vi "calculate_wildcard_filename_from_sibling_filenames.vi"(10 "shared library filename":string, 11 "sibling filenames":string[](array[string])) -> (2 "wildcard filename":string, 3 "sibling shared libraries":string[](array[string]))   [LabVIEW 2020, in "vi_package_building_extensions.lvlib" / "fix_shared_library_wildcards.lvlib"]
uses:
  fix_shared_library_wildcards.lvlib
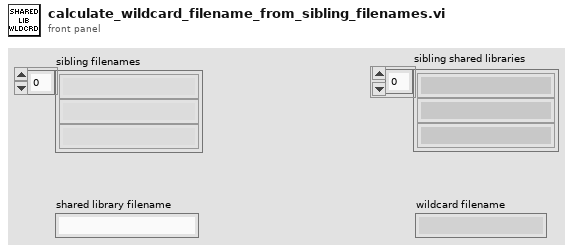
[diagram p1: front panel]
types:
  T1 = cluster{"search regex":string, "replacement":string}
  T2 = cluster{"search regex":string, "replacement":string}[]
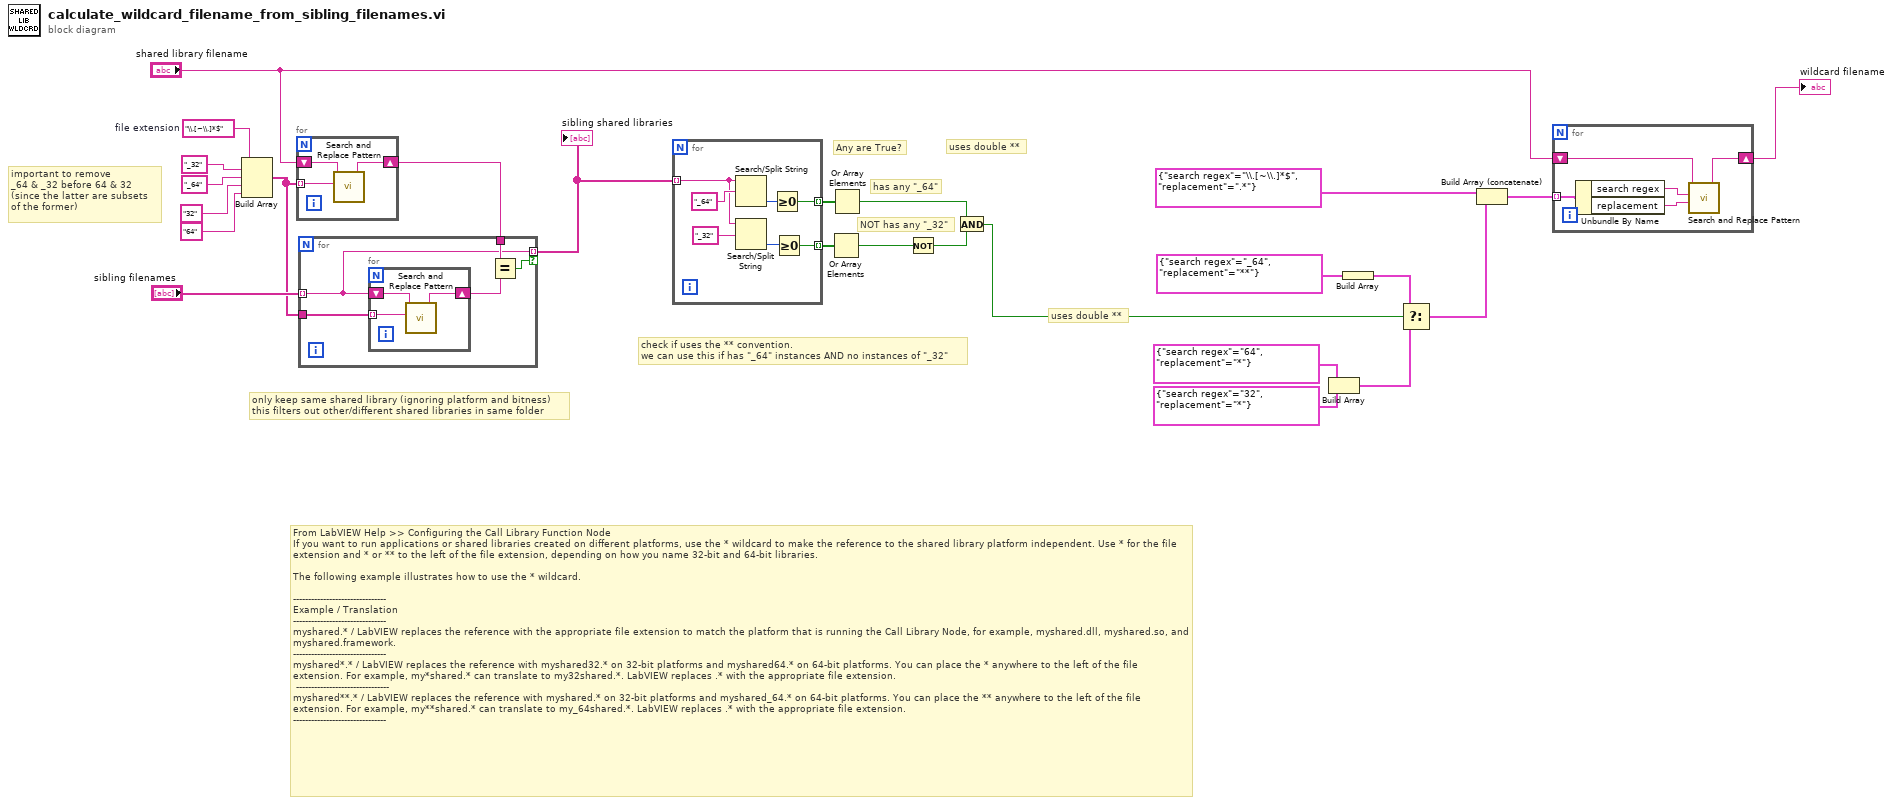
[diagram p0: block diagram]
diagram:
  w20 = "\\.[~\\.]*$"  # file extension
  # "From LabVIEW Help >> Configuring the Call Library Function Node\nIf you want to run applications or shared libraries created on different platforms, use the * wildcard to make the reference to the shared library platform independent. Use * for the file extension and * or ** to the left of the file extension, depending on how you name 32-bit and 64-bit libraries.\n\nThe following example illustrates how to use the * wildcard.\n\n-------------------------------\nExample / Translation\n-------------------------------\nmyshared.* / LabVIEW replaces the reference with the appropriate file extension to match the platform that is running the Call Library Node, for example, myshared.dll, myshared.so, and myshared.framework. \n-------------------------------\nmyshared*.* / LabVIEW replaces the reference with myshared32.* on 32-bit platforms and myshared64.* on 64-bit platforms. You can place the * anywhere to the left of the file extension. For example, my*shared.* can translate to my32shared.*. LabVIEW replaces .* with the appropriate file extension.\n -------------------------------\nmyshared**.* / LabVIEW replaces the reference with myshared.* on 32-bit platforms and myshared_64.* on 64-bit platforms. You can place the ** anywhere to the left of the file extension. For example, my**shared.* can translate to my_64shared.*. LabVIEW replaces .* with the appropriate file extension. \n-------------------------------"
  # "uses double **"
  # "only keep same shared library (ignoring platform and bitness)\nthis filters out other/different shared libraries in same folder"
  # "important to remove\n_64 & _32 before 64 & 32 (since the latter are subsets of the former)"
  # "check if uses the ** convention.\nwe can use this if has \"_64\" instances AND no instances of \"_32\""
  # "uses double **"
  # "NOT has any \"_32\""
  # "has any \"_64\""
  # "Any are True?"
  n1 = Build Array(w20, "_32", "_64", "32", "64") -> (w15:string[])
  n2 = for {
    tunnel: w15 -> [w28] mode=indexing
    shift-right: [w26] -> w14
    shift-left: "shared library filename" -> [w27]
    n3 = call <vilib>:"Search and Replace Pattern.vi"("string"=w27, "regular expression (\"\")"=w28) -> ("result string"=w26:string)  [unwired: 3 in, 1 out]
  }
  n4 = for {
    tunnel: "sibling filenames" -> [w30] mode=indexing
    tunnel: w15 -> [w33]
    tunnel: w14 -> [w32]
    tunnel: [w30] -> w13 mode=indexing if=w31
    n5 = for {
      tunnel: w33 -> [w36] mode=indexing
      shift-right: [w34] -> w29
      shift-left: w30 -> [w35]
      n6 = call <vilib>:"Search and Replace Pattern.vi"("string"=w35, "regular expression (\"\")"=w36) -> ("result string"=w34:string)  [unwired: 3 in, 1 out]
    }
    n7 = Equal?(x=w32, y=w29) -> (x = y?=w31:bool)
  }
  "sibling shared libraries" <- w13
  n8 = for {
    tunnel: w13 -> [w41] mode=indexing
    tunnel: [w37] -> w24 mode=indexing
    tunnel: [w38] -> w25 mode=indexing
    n9 = Search/Split String(string=w41, search string/char (-)="_64") -> (offset of match=w40:i32)  [unwired: 1 in, 2 out]
    n10 = Search/Split String(string=w41, search string/char (-)="_32") -> (offset of match=w39:i32)  [unwired: 1 in, 2 out]
    n11 = Greater Or Equal To 0?(x=w40) -> (x >= 0?=w37:bool)
    n12 = Greater Or Equal To 0?(x=w39) -> (x >= 0?=w38:bool)
  }
  n13 = Or Array Elements(Boolean array=w25) -> (logical OR=w23:bool)
  n14 = Or Array Elements(Boolean array=w24) -> (logical OR=w22:bool)
  n15 = Not(x=w23) -> (.not. x?=w21:bool)
  n16 = And(x=w22, y=w21) -> (x .and. y?=w7:bool)
  n17 = Build Array(T1 {"search regex"="64", "replacement"="*"}, T1 {"search regex"="32", "replacement"="*"}) -> (w8:T2)
  n18 = Build Array(T1 {"search regex"="_64", "replacement"="**"}) -> (w9:T2)
  n19 = Select(t=w9, s=w7, f=w8) -> (s? t:f=w5:T2)
  n20 = Build Array (concatenate)(T1 {"search regex"="\\.[~\\.]*$", "replacement"=".*"}, w5) -> (w2:T2)
  n21 = for {
    shift-right: [w47] -> w4
    shift-left: "shared library filename" -> [w48]
    tunnel: w2 -> [w46] mode=indexing
    n22 = Unbundle By Name(w46) -> ("search regex"=w45:string, "replacement"=w44:string)
    n23 = call <vilib>:"Search and Replace Pattern.vi"("string"=w48, "regular expression (\"\")"=w45, "replace string (\"\")"=w44) -> ("result string"=w47:string)  [unwired: 2 in, 1 out]
  }
  "wildcard filename" <- w4
